vi "NR set HO Param.vi"(7 "Operation Band":u32, 8 "error in (no error)":errorcluster caption="에러 입력(에러 없음)", 9 "Center Channel Number":u32, 10 "BW (MHz)":u32, 11 "Instrument Manager 입력":refnum<class "Instrument Manager.lvclass">) -> (0 "error out":errorcluster caption="에러 출력", 3 "Instrument Manager 출력":refnum<class "Instrument Manager.lvclass">)   [LabVIEW 2023, in "Instrument Manager.lvclass"]
uses:
  Instrument Manager.lvclass
  Instrument Manager.lvclass/Instrument Manager.ctl
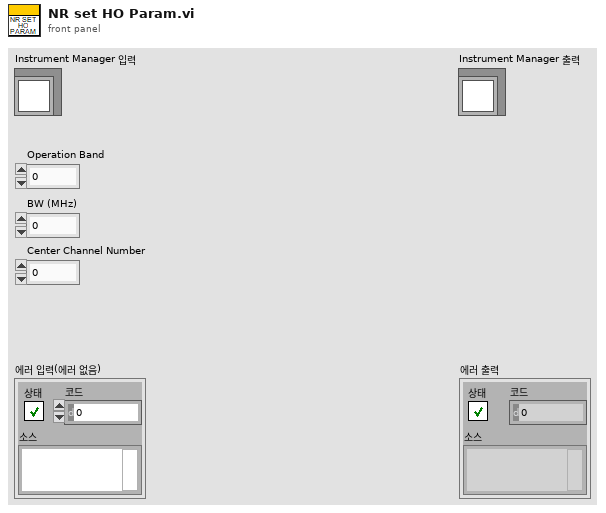
[diagram p1: front panel]
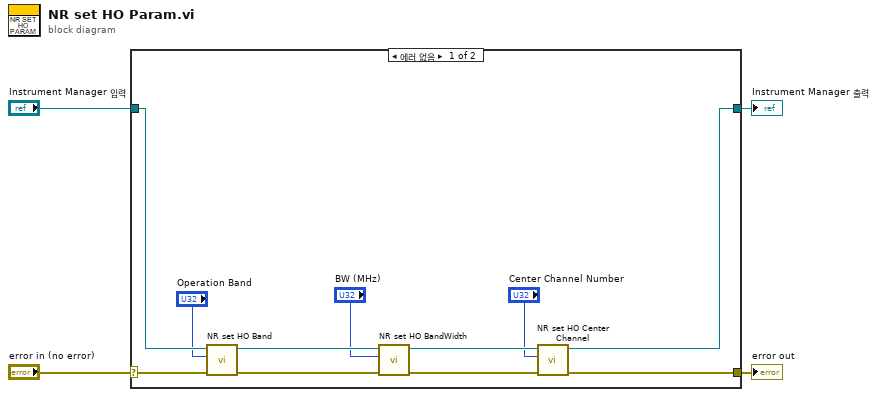
[diagram p0: block diagram]
diagram:
  n1 = case shown="에러 없음" "error in (no error)" {
    selector: "error in (no error)" -> [w15 w17]
    tunnel: [w12 w17] -> w3
    tunnel: [w8 w16] -> w1
    tunnel: "Instrument Manager 입력" -> [w11 w16]
    frame No Error {
      n2 = call "NR set HO Band.vi"("error in (no error)"=w15, "Operation Band"="Operation Band", "Instrument Manager 입력"=w11) -> ("error out"=w14:errorcluster, "Instrument Manager 출력"=w10:refnum<class "Instrument Manager.lvclass">)  [unwired: 7 in]
      n3 = call "NR set HO BandWidth.vi"("error in (no error)"=w14, "BW (MHz)"="BW (MHz)", "Instrument Manager 입력"=w10) -> ("error out"=w13:errorcluster, "Instrument Manager 출력"=w9:refnum<class "Instrument Manager.lvclass">)  [unwired: 7 in]
      n4 = call "NR set HO Center Channel.vi"("error in (no error)"=w13, "Center Channel Number"="Center Channel Number", "Instrument Manager 입력"=w9) -> ("error out"=w12:errorcluster, "Instrument Manager 출력"=w8:refnum<class "Instrument Manager.lvclass">)  [unwired: 7 in]
    }
    frame Error {
    }
  }
  "error out" <- w3
  "Instrument Manager 출력" <- w1
